vi "KYFG Buffer Delete.vi"(8 "error in (no error)":errorcluster, 11 "streamHandle":u32) -> (0 "error out":errorcluster)   [LabVIEW 2023, in "KYFGLib_lv.lvlib"]
doc: "KYFG_API FGSTATUS KYFG_BufferDelete(BUFFHANDLE buffHandle);"
uses:
  KYFGLib_lv.lvlib
  KYFGLib.dll
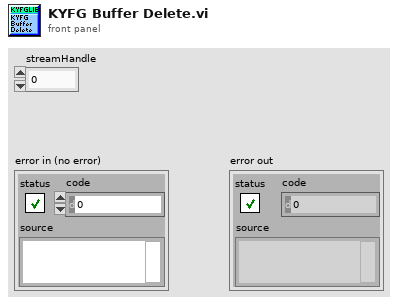
[diagram p1: front panel]
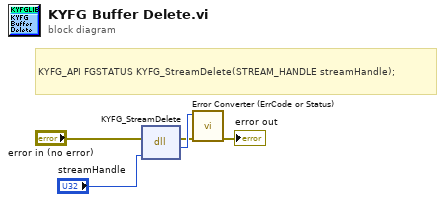
[diagram p0: block diagram]
diagram:
  # "KYFG_API FGSTATUS\tKYFG_StreamDelete(STREAM_HANDLE streamHandle);"
  n1 = dll-call lib="KYFGLib.dll" fn="KYFG_StreamDelete"(error in="error in (no error)", "streamHandle"="streamHandle") -> (error out=w2:errorcluster, "return type"=w5:u32)  [unwired: 3 in, 1 out]
  n2 = call "Error Converter (ErrCode or Status).vi"("error in (no error)"=w2, "error code"=w5) -> ("error out"=→"error out":errorcluster)  [unwired: 9 in]
